vi "VI Tree.vi"() -> ()   [LabVIEW 2017]
uses:
  Private/RegisterVI.vi
  Private/RegisterVIs.vi
  API/JKI Simple Localization.lvlib
panel:
  out "OS Primary Language":string
  out "Languages":string[](array[string])
  out "Languages":string[](array[string])
  out "Translated Phrase":string
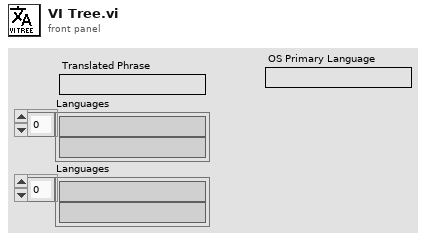
[diagram p1: front panel]
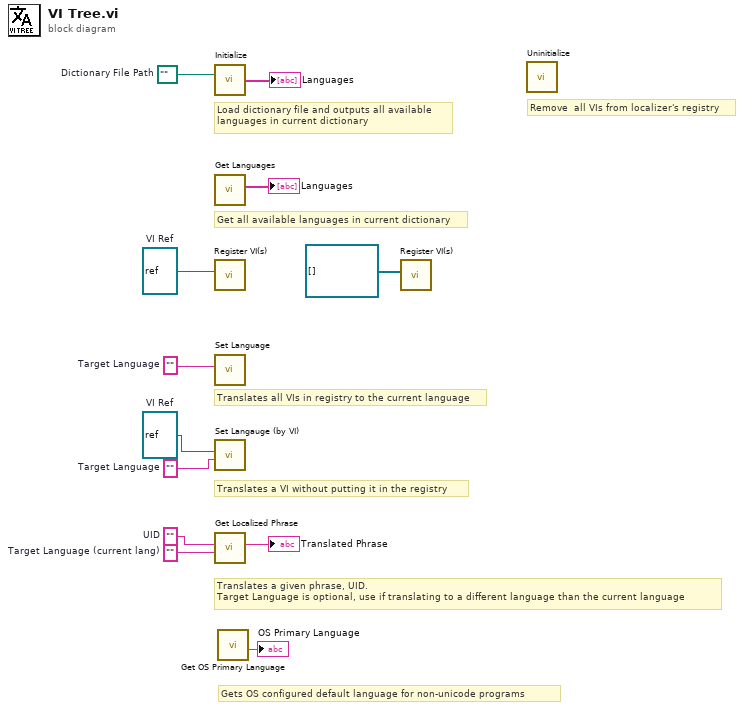
[diagram p0: block diagram]
diagram:
  w2 = ""  # Target Language
  w3 = ""  # Target Language
  w4 = refnum<vi> refnum  # VI Ref
  w5 = path ""  # Dictionary File Path
  w11 = ""  # Target Language (current lang)
  w10 = ""  # UID
  w8 = refnum<vi> refnum  # VI Ref
  # "Gets OS configured default language for non-unicode programs"
  # "Translates a VI without putting it in the registry"
  # "Remove  all VIs from localizer's registry"
  # "Translates a given phrase, UID.\nTarget Language is optional, use if translating to a different language than the current language"
  # "Translates all VIs in registry to the current language"
  # "Get all available languages in current dictionary"
  # "Load dictionary file and outputs all available languages in current dictionary"
  n1 = call "Initialize.vi"("Dictionary File Path"=w5) -> ("Languages"=→"Languages":string[])  [unwired: 11 in, 3 out]
  n2 = call "Get Languages.vi"() -> ("Languages"=→"Languages":string[])  [unwired: 10 in, 1 out]
  n3 = call-poly "Register VI(s).vi"("VI Ref"=w8) -> ()  [unwired: 9 in, 2 out]
  n4 = call "Set Language.vi"("Target Language (current lang)"=w2) -> ()  [unwired: 9 in, 2 out]
  n5 = call "Set Langauge (by VI).vi"("Target Language"=w3, "VI Ref"=w4) -> ()  [unwired: 9 in, 1 out]
  n6 = call "Get Localized Phrase.vi"("Target Language (current lang)"=w11, "Key"=w10) -> ("Translated Phrase"=→"Translated Phrase":string)  [unwired: 8 in, 1 out]
  n7 = call "Get OS Primary Language.vi"() -> ("OS Primary Language"=→"OS Primary Language":string)  [unwired: 10 in, 1 out]
  n8 = call-poly "Register VI(s).vi"("VI References"=refnum<vi>[] []) -> ()  [unwired: 9 in, 2 out]
  n9 = call "Uninitialize.vi"() -> ()  [unwired: 11 in, 1 out]
